vi "vi_bd.vi"() -> ()   [LabVIEW 2014]
panel:
  out "Block Diagram":refnum<vi>
  out "error out":errorcluster
  out "reference out":refnum<vi>
  in  "error in (no error)":errorcluster
  in  "reference":refnum<vi>
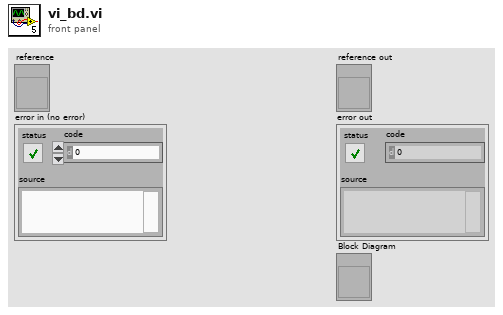
[diagram p1: front panel]
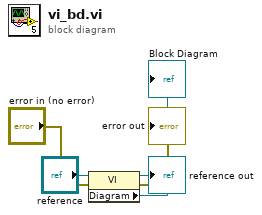
[diagram p0: block diagram]
diagram:
  n1 = property class="VI"(reference="reference", error in="error in (no error)") -> (reference out=→"reference out":refnum<vi>, error out=→"error out":errorcluster, "Diagram"=→"Block Diagram":refnum<vi>)
